vi "operation_func.vi"(9 "INPUT in":dbl, 10 "INPUT 1":dbl, 11 "MENU OPTION":T1(ring)) -> (2 "Numeric":dbl, 3 "Boolean":bool)   [LabVIEW 2016]
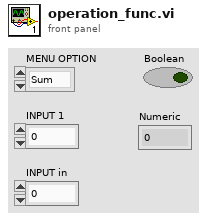
[diagram p1: front panel]
types:
  T1 = enum16{"Sum", "Divide", "Substract", "Multiplpy"}
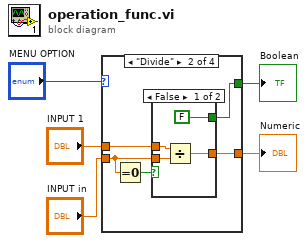
[diagram p0: block diagram]
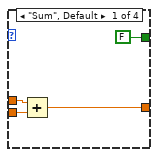
[diagram p2: hidden frame]
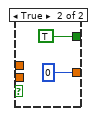
[diagram p3: hidden frame]
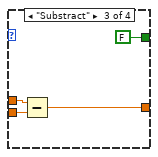
[diagram p4: hidden frame]
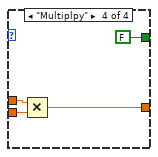
[diagram p5: hidden frame]
diagram:
  n1 = case shown="\"Divide\"" "MENU OPTION" {
    tunnel: [FALSE w14 FALSE FALSE] -> w2
    tunnel: "INPUT 1" -> [w8 w11 w23 w27]
    tunnel: "INPUT in" -> [w7 w10 w22 w26]
    tunnel: [w6 w12 w24 w28] -> w5
    frame "Sum", Default {
      n2 = Add(x=w8, y=w7) -> (x+y=w6:dbl)
    }
    frame "Divide" {
      n3 = Equal To 0?(x=w10) -> (x = 0?=w13:bool)
      n4 = case shown="False" w13 {
        tunnel: [FALSE TRUE] -> w14
        tunnel: [w17 0] -> w12
        tunnel: w11 -> [w16 _]
        tunnel: w10 -> [w15 _]
        frame False {
          n5 = Divide(x=w16, y=w15) -> (x/y=w17:dbl)
        }
        frame True {
        }
      }
    }
    frame "Substract" {
      n6 = Subtract(x=w23, y=w22) -> (x-y=w24:dbl)
    }
    frame "Multiplpy" {
      n7 = Multiply(x=w27, y=w26) -> (x*y=w28:dbl)
    }
  }
  "Numeric" <- w5
  "Boolean" <- w2
